vi "8-Tap 8-bit Camera with DRAM Modified (Host).vi"() -> ()   [LabVIEW 2013]
doc: "This is the host VI for the 10-Tap 8-Bit Camera with DRAM example. This example demonstrates how to acquire images from a 10-tap, 8-bit, extended configuration, Camera Link camera and display the images on the host. This example supports area scan and line scan cameras for both continuous and finite acquisitions.\n\nThis example also demonstrates the use of DRAM as a frame buffer for very high speed acquisitions. Data packing and flow-control are also employed to maximize use of the available DRAM and FIFOs in terms of both memory space and performance.\n\nAdditionally, the example demonstrates the serial server, which allows third-party camera configuration utilities to communicate with the camera using the Camera Link serial interface while this VI is running."
uses:
  <vilib>/userdefined/High Color/nirio_resource_hc.ctl
  <vilib>/rvi/interface/common/niFpgaWaitOnOcc.vi
  <vilib>/FPGAPlugInAG/PCIe-1473R/niLvFpga_Reset_PCIe-1473R.vi
  <vilib>/Utility/error.llb/Error Cluster From Error Code.vi
  <vilib>/rvi/errors/niLvFpgaAdjustHostInterfaceError.vi
  <vilib>/FPGAPlugInAG/PCIe-1473R/niLvFpga_Run_PCIe-1473R.vi
  <vilib>/FPGAPlugInAG/PCIe-1473R/niLvFpga_Close_PCIe-1473R.vi
  <vilib>/rvi/interface/nirviMethod/nirviMethod.xnode
  Host/FGs/FPGA_Reference.ctl
  FPGA Bitfiles/8-Tap8-bitCamera_FPGATarget_8-Tap8-bit_Serial_Server.lvbitx
  <vilib>/rvi/interface/nirviReadWriteControl/nirviReadWriteControl.xnode
  Common/CL Configuration.ctl
  Common/CL Signal Mapping.ctl
  <vilib>/rvi/interface/nirviCloseFPGA/nirviCloseFPGA.xnode
  NiFpgaLv.dll
  <vilib>/rvi/errors/niLvFpgaMergeErrorWithErrorCode.vi
  <vilib>/FPGAPlugInAG/PCIe-1473R/niLvFpga_ConfigureFifo_PCIe-1473R.vi
  <vilib>/FPGAPlugInAG/PCIe-1473R/niLvFpga_StartFifo_PCIe-1473R.vi
  <vilib>/FPGAPlugInAG/PCIe-1473R/niLvFpga_ReadFifo_PCIe-1473R.vi
panel:
  out "Elements Remaining":u32
  in  "DMA Buffer Size\n(In Images)":u32=2200 caption="DMA Buffer Size"
  in  "Signal Mapping":T1(ring)
  out "Acq In Progress":bool
  in  "Line Scan":bool
  in  "Frames To Acquire":u32 caption="Frames To Acquire\n(0 = infinite)"
  in  "Cancel":bool
  out "Acq'd Frame Width":u32=1200
  in  "Stopped":bool=TRUE
  in  "RIO Device":T2="RIO0"
  out "DMA Write Timeout":bool
  in  "Start Serial Server":bool=TRUE
  out "Frames Acq'd":u32=593
  out "Acq'd Frame Height":u32=788
  out "Image":T3(plugin-control)
  in  "Acquire":bool
  in  "Stop":bool
  in  "Image Height":u32=788 max=65535
  in  "Image Width":u32=1200 max=65535 step=40
  out "Initialized":bool
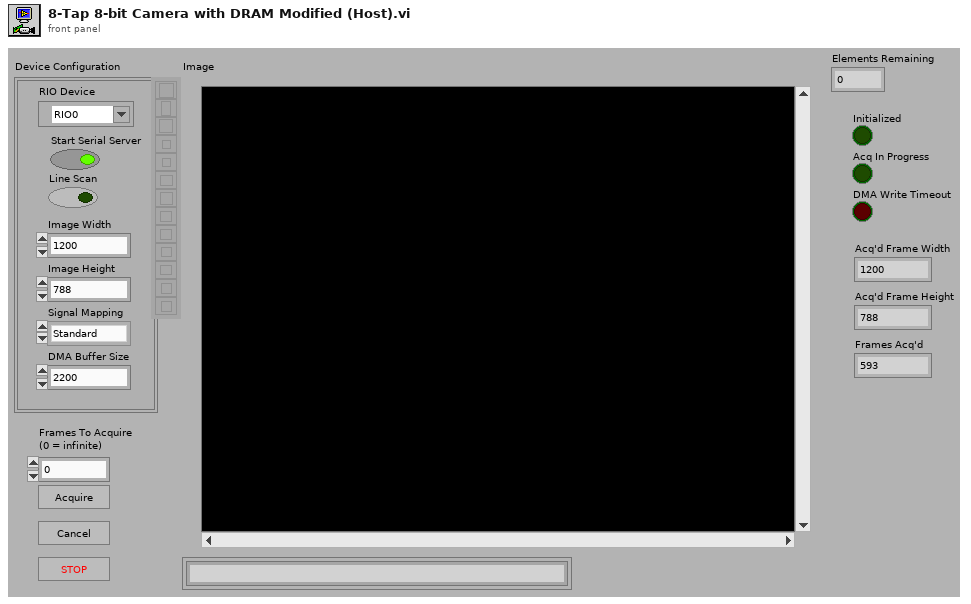
[diagram p1: front panel]
types:
  T1 = enum8{"Standard", "Basler 10-tap", "Vosskühler 10-tap"}
  T2 = typedef "nirio_resource_hc.ctl" = tag
  T3 = typedef "IMAQ Image.ctl" = refnum<image>
  T4 = typedef "Image Type" = u32
  T5 = typedef "FPGA_Reference.ctl" = refnum<k20>
  T6 = enum16{"big-endian, network order", "native, host order", "little-endian"}
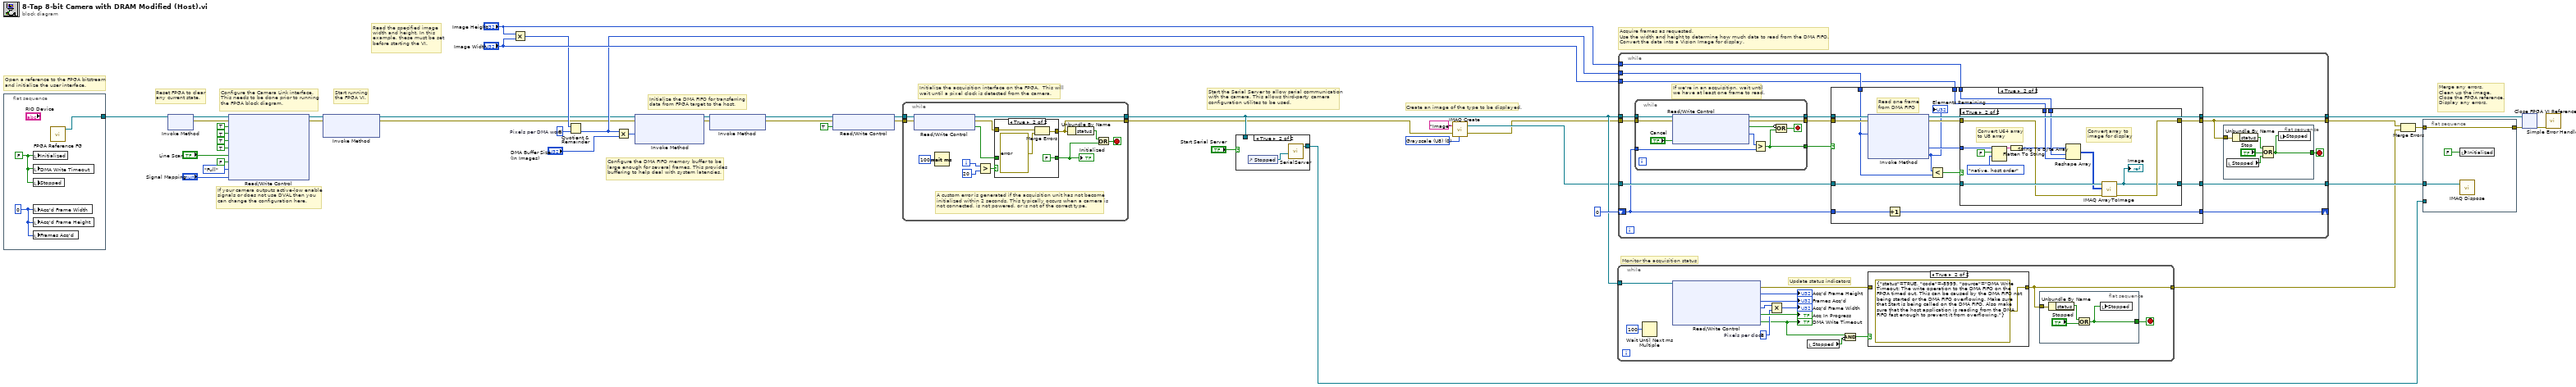
[diagram p0: block diagram]
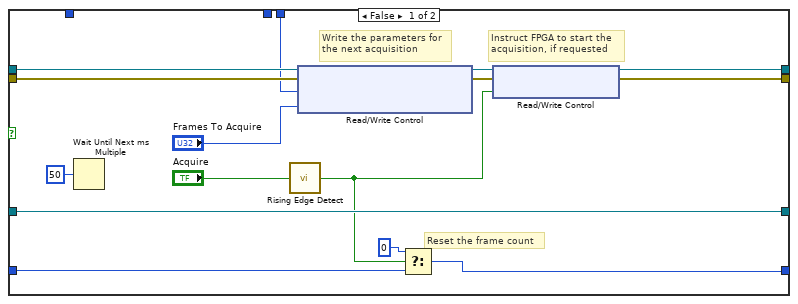
[diagram p4: hidden frame]
diagram:
  w5 = u32 8  # Pixels per DMA word
  w42 = T4 0 items=["Grayscale (U8)", "Grayscale (I16)", "Grayscale (SGL)", "Complex (CSG)", "RGB (U32)", "HSL (U32)", "RGB (U64)", "Grayscale (U16)"] ("Image Type")
  # "If your camera outputs active-low enable\nsignals or does not use DVAL then you \ncan change the configuration here."
  # "Configure the DMA FIFO memory buffer to be\nlarge enough for several frames. This provides\nbuffering to help deal with system latencies."
  # "Start running\nthe FPGA VI."
  # "Reset FPGA to clear\nany current state."
  # "Read the specified image\nwidth and height. In this\nexample, these must be set\nbefore starting the VI."
  # "Merge any errors.\nClean up the image.\nClose the FPGA reference.\nDisplay any errors."
  # "Acquire frames as requested.\nUse the width and height to determine how much data to read from the DMA FIFO.\nConvert the data into a Vision Image for display."
  # "Monitor the acquisition status"
  # "Start the Serial Server to allow serial communication\nwith the camera. This allows third-party camera\nconfiguration utilites to be used."
  # "Create an image of the type to be displayed."
  # "Initialize the acquisition interface on the FPGA.  This will\nwait until a pixel clock is detected from the camera."
  # "Initialize the DMA FIFO for transferring\ndata from FPGA target to the host."
  # "Configure the Camera Link interface.\nThis needs to be done prior to running\nthe FPGA block diagram."
  # "Open a reference to the FPGA bitstream\nand initialize the user interface."
  n1 = flat-sequence {
    tunnel: [w46] -> w33
    frame #0 {
      w48 = u32 0 ("Num Lines Acq'd")
      w47 = FALSE ("stop")
      n2 = local write "Initialized"(w47) -> ()
      n3 = local write "DMA Write Timeout"(w47) -> ()
      n4 = local write "Stopped"(w47) -> ()
      n5 = local write "Acq'd Frame Width"(w48) -> ()
      n6 = local write "Acq'd Frame Height"(w48) -> ()
      n7 = local write "Frames Acq'd"(w48) -> ()
      n8 = call "FPGA Reference FG.vi"() -> ("FPGA VI Reference Out"=w46:T5)  [unwired: 11 in]
    }
  }
  n9 = xnode "Invoke Method"("FPGA VI Reference In"=w33) -> ("FPGA VI Reference Out"=w22:T5, "error out"=w25:errorcluster)  [unwired: 1 in]
  n10 = xnode "Read/Write Control"("FPGA VI Reference In"=w22, "error in"=w25, "CL Config.FVAL Active High"=TRUE ("IO Module Config.CL FVAL Active High"), "CL Config.LVAL Active High"=TRUE ("IO Module Config.CL LVAL Active High"), "CL Config.DVAL Active High"=TRUE ("IO Module Config.CL DVAL Active High"), "CL Config.Spare Active High"=TRUE ("IO Module Config.CL Spare Active High"), "CL Config.Line Scan"="Line Scan", "Acq Control.Ignore DVAL"=FALSE ("CL Config.Line Scan"), "CL Config.Configuration"=enum8{"Base", "Medium", "Full"}."Full", "CL Config.Signal Mapping"="Signal Mapping") -> ("FPGA VI Reference Out"=w26:T5, "error out"=w24:errorcluster)
  n11 = xnode "Invoke Method"("FPGA VI Reference In"=w26, "error in"=w24) -> ("FPGA VI Reference Out"=w2:T5, "error out"=w1:errorcluster)  [unwired: 1 in]
  n12 = Multiply(x="Image Height", y="Image Width") -> (x*y=w4:u32)
  n13 = Quotient & Remainder(x=w4, y=w5) -> (floor(x/y)=w3:u32)  [unwired: 1 out]
  n14 = Multiply(x=w3, y="DMA Buffer Size\n(In Images)") -> (x*y=w16:u32)
  n15 = xnode "Invoke Method"("FPGA VI Reference In"=w2, "error in"=w1, "Requested Depth"=w16) -> ("FPGA VI Reference Out"=w32:T5, "error out"=w31:errorcluster)  [unwired: 1 out]
  n16 = xnode "Invoke Method"("FPGA VI Reference In"=w32, "error in"=w31) -> ("FPGA VI Reference Out"=w17:T5, "error out"=w30:errorcluster)
  n17 = xnode "Read/Write Control"("FPGA VI Reference In"=w17, "error in"=w30, "Acq Control.Initialize"=TRUE ("Arm Acquisition")) -> ("FPGA VI Reference Out"=w45:T5, "error out"=w44:errorcluster)
  n18 = while {
    tunnel: w45 -> [w56]
    tunnel: w44 -> [w55]
    tunnel: [w54] -> w13
    tunnel: [w58] -> w12
    i -> [w50]
    stop <- w61 stop-if-true
    # "A custom error is generated if the acquisition unit has not become\ninitialized within 2 seconds. This typically occurs when a camera is\nnot connected, is not powered, or is not of the correct type."
    n19 = xnode "Read/Write Control"("FPGA VI Reference In"=w56, "error in"=w55) -> ("FPGA VI Reference Out"=w54:T5, "error out"=w53:errorcluster, "Acq Status.Initialized"=w52:bool)
    n20 = Wait (ms)(milliseconds to wait=u32 100) -> ()  [unwired: 1 out]
    n21 = Greater?(x=w50, y=20) -> (0:w51:bool)
    n22 = case shown="True" w51 {
      tunnel: [w63 FALSE] -> w57
      tunnel: w52 -> [w63 _]
      tunnel: w53 -> [w62 w65]
      tunnel: [w62 w67] -> w58
      frame False {
      }
      frame True {
        n23 = Merge Errors(w65, errorcluster {"status"=TRUE, "code"=-8999, "source"="Acquisition Initialization: This error typically occurs when a camera is not properly connected, is not powered, or is not of the correct type."} ("error in")) -> (w67:errorcluster)
      }
    }
    "Initialized" <- w57
    n24 = Unbundle By Name(w58) -> ("status"=w60:bool)
    n25 = Or(x=w60, y=w57) -> (x .or. y?=w61:bool)
  }
  n26 = case shown="True" "Start Serial Server" {
    tunnel: [_ w68] -> w34
    tunnel: w13 -> [_ _]
    frame False {
    }
    frame True {
      n27 = control-ref of="Stopped"() -> (w69:refnum<vi>)
      n28 = call "SerialServer.vi"("Stop Refnum"=w69) -> ("FPGA VI Reference Out"=w68:refnum<k20>)  [unwired: 6 in]
    }
  }
  n29 = call "IMAQ Create"("Image Name"="Image", "Image Type"=w42, "error in (no error)"=w12) -> ("New Image"=w9:T3, "error out"=w8:errorcluster)  [unwired: 2 in]
  n30 = while {
    tunnel: w13 -> [w80]
    tunnel: [w83] -> w27
    stop <- w82 stop-if-true
    w73 = u32 8  # Pixels per clock
    # "Update status indicators"
    n31 = Wait Until Next ms Multiple(millisecond multiple=u32 100) -> ()  [unwired: 1 out]
    n32 = xnode "Read/Write Control"("FPGA VI Reference In"=w80) -> ("error out"=w79:errorcluster, "Acq Status.Lines Per Frame"=→"Acq'd Frame Height":u32, "Acq Status.Frames Acq'd"=→"Frames Acq'd":u32, "Acq Status.Clocks Per Line"=w74:u32, "Acq Status.Acq In Progress"=→"Acq In Progress":bool, "Acq Status.DMA Write Timeout"=w71:bool)  [unwired: 1 in, 1 out]
    "DMA Write Timeout" <- w71
    n33 = Multiply(x=w74, y=w73) -> (x*y=→"Acq'd Frame Width":u32)
    n34 = local read "Stopped"() -> (w70:bool)
    n35 = Compound Arithmetic op=AND(w71, invert w70) -> (w72:bool)
    n36 = case shown="True" w72 {
      tunnel: w79 -> [w88 _]
      tunnel: [w88 errorcluster {"status"=TRUE, "code"=-8999, "source"="DMA Write Timeout: The write operation to the DMA FIFO on the FPGA timed out. This can be caused by the DMA FIFO not being started or the DMA FIFO overflowing. Make sure that Start is being called on the DMA FIFO. Also make sure that the host application is reading from the DMA FIFO fast enough to prevent it from overflowing."} ("error out")] -> w83
      frame False {
      }
      frame True {
      }
    }
    n37 = flat-sequence {
      tunnel: w83 -> [w87]
      tunnel: [w85] -> w82
      frame #0 {
        n38 = Unbundle By Name(w87) -> ("status"=w86:bool)
        n39 = Or(x=w86, y="Stopped") -> (x .or. y?=w85:bool)
        n40 = local write "Stopped"(w85) -> ()
      }
    }
  }
  n41 = while {
    tunnel: w13 -> [w96]
    tunnel: w8 -> [w95]
    tunnel: w3 -> [w104]
    tunnel: "Image Height" -> [w103]
    tunnel: "Image Width" -> [w102]
    tunnel: w9 -> [w101]
    tunnel: [w99] -> w28
    tunnel: [w100] -> w41
    tunnel: [w97] -> w36
    shift-right: [w91] -> _
    shift-left: u32 0 -> [w90]
    stop <- w98 stop-if-true
    # "If we're in an acquisition, wait until\nwe have at least one frame to read."
    n42 = while {
      tunnel: w96 -> [w111]
      tunnel: w95 -> [w110]
      tunnel: [w108] -> w94
      tunnel: [w109] -> w93
      tunnel: w90 -> [w114]
      tunnel: [w112] -> w92
      stop <- w113 stop-if-true
      n43 = xnode "Read/Write Control"("FPGA VI Reference In"=w111, "error in"=w110, "Acq Control.Cancel Acq"="Cancel") -> ("FPGA VI Reference Out"=w109:T5, "error out"=w108:errorcluster, "Acq Status.Acq In Progress"=w107:bool, "Acq Status.Frames Acq'd"=w106:u32)
      n44 = Greater?(x=w106, y=w114) -> (0:w112:bool)
      n45 = Compound Arithmetic op=OR(invert w107, w112) -> (w113:bool)
    }
    n46 = case shown="True" w92 {
      tunnel: w93 -> [w130 w142]
      tunnel: w94 -> [w129 w141]
      tunnel: w104 -> [_ w135]
      tunnel: w103 -> [w123 w149]
      tunnel: w102 -> [_ w148]
      tunnel: w101 -> [w134 w147]
      tunnel: [w125 w145] -> w99
      tunnel: [w128 w144] -> w100
      tunnel: [w134 w143] -> w97
      tunnel: w90 -> [w131 w140]
      tunnel: [w133 w139] -> w91
      frame False {
        # "Reset the frame count"
        # "Instruct FPGA to start the\nacquisition, if requested"
        # "Write the parameters for\nthe next acquisition"
        n47 = Wait Until Next ms Multiple(millisecond multiple=u32 50) -> ()  [unwired: 1 out]
        n48 = call "Rising Edge Detect.vi"("Input"="Acquire") -> ("Pulse"=w120:bool)  [unwired: 4 in]
        n49 = xnode "Read/Write Control"("FPGA VI Reference In"=w130, "error in"=w129, "Acq Control.Line Scan Height"=w123, "Acq Control.Frames To Acq"="Frames To Acquire") -> ("FPGA VI Reference Out"=w127:T5, "error out"=w126:errorcluster)
        n50 = Select(t=u32 0, s=w120, f=w131) -> (s? t:f=w133:u32)
        n51 = xnode "Read/Write Control"("FPGA VI Reference In"=w127, "error in"=w126, "Acq Control.Acquire"=w120) -> ("FPGA VI Reference Out"=w128:T5, "error out"=w125:errorcluster)
      }
      frame True {
        # "Read one frame\nfrom DMA FIFO"
        n52 = xnode "Invoke Method"("FPGA VI Reference In"=w142, "error in"=w141, "Number of Elements"=w135) -> ("FPGA VI Reference Out"=w144:T5, "error out"=w146:errorcluster, "Data"=w138:u64[], "Elements Remaining"=w136:u32)  [unwired: 1 in]
        "Elements Remaining" <- w136
        n53 = Increment(x=w140) -> (x+1=w139:u32)
        n54 = Less?(x=w136, y=w135) -> (x < y?=w137:bool)
        n55 = case shown="True" w137 {
          tunnel: w149 -> [_ w163]
          tunnel: w148 -> [_ w162]
          tunnel: w147 -> [w151 w161]
          tunnel: w146 -> [w150 w160]
          tunnel: [w150 w159] -> w145
          tunnel: [w151 w158] -> w143
          tunnel: w138 -> [_ w155]
          frame False {
            # "Do not display the image if we're falling behind in the acquisition."
          }
          frame True {
            # "Convert U64 array\nto U8 array"
            # "Convert array to\nimage for display"
            n56 = Flatten To String(anything=w155, prepend array or string size? (T)=FALSE, byte order (0:big-endian, network order)=T6."native, host order") -> (data string=w153:string)  [unwired: 1 in, 2 out]
            n57 = String To Byte Array(string=w153) -> (unsigned byte array=w152:u8[])
            n58 = Reshape Array(w152, w163, w162) -> (w157:u8[][])
            n59 = call "IMAQ ArrayToImage"("error in (no error)"=w160, "Image Pixels (U8)"=w157, "Image"=w161) -> ("error out"=w159:errorcluster, "Image Out"=w158:T3)  [unwired: 7 in]
            "Image" <- w158
          }
        }
      }
    }
    n60 = flat-sequence {
      tunnel: w99 -> [w117]
      tunnel: [w116] -> w98
      frame #0 {
        n61 = local read "Stopped"() -> (w115:bool)
        n62 = Unbundle By Name(w117) -> ("status"=w118:bool)
        n63 = Compound Arithmetic op=OR(w118, "Stop", w115) -> (w116:bool)
        n64 = local write "Stopped"(w116) -> ()
      }
    }
  }
  n65 = Merge Errors(w28, w27) -> (w29:errorcluster)
  n66 = flat-sequence {
    tunnel: w29 -> [w165]
    tunnel: [w165] -> w38
    tunnel: w36 -> [w166]
    tunnel: w34 -> [_]
    frame #0 {
      n67 = local write "Initialized"(FALSE ("Module Enabled")) -> ()
      n68 = call "IMAQ Dispose"("Image"=w166) -> ()  [unwired: 5 in, 1 out]
    }
  }
  n69 = xnode "Close FPGA VI Reference"("FPGA VI Reference In"=w41, "error in"=w38) -> ("error out"=w35:errorcluster)
  n70 = call <vilib>:"Simple Error Handler.vi"("error in (no error)"=w35) -> ()  [unwired: 4 in, 5 out]
